vi "base ex info array formation.vi"(11 "Ex info":T1) -> (0 "Tag":string, 1 "Tag 2":string, 3 "Base Ex info array":string[](array[string]))   [LabVIEW 2018]
panel:
  out "配列":string[](array[string])
  out "文字列":string
  out "Level Composition":string[](array[string])
  out "サイズ":i32
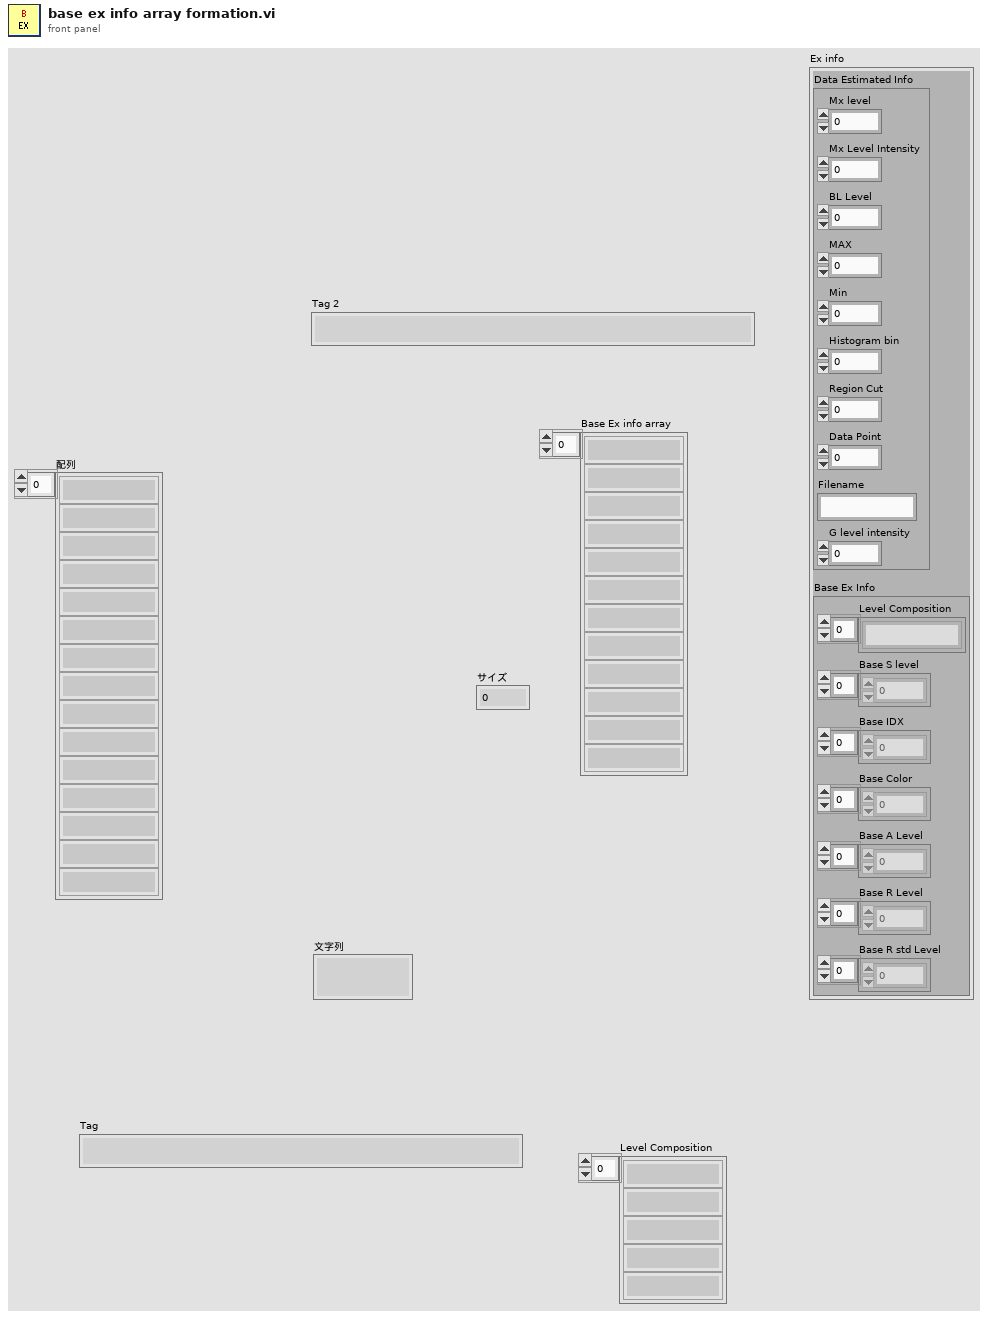
[diagram p1: front panel]
types:
  T1 = cluster{"Data Estimated Info":cluster{"Mx level":dbl, "Mx Level Intensity":dbl, "BL Level":dbl, "MAX":dbl, "Min":dbl, "Histogram bin":dbl, "Region Cut":dbl, "Data Point":i32, "Filename":string, "G level intensity":dbl}, "Base Ex Info":cluster{"Level Composition":string[], "Base S level":dbl[], "Base IDX":i32[], "Base Color":u32[], "Base A Level":dbl[], "Base R Level":dbl[], "Base R std Level":dbl[]}}
  T2 = cluster{"Mx level":dbl, "Mx Level Intensity":dbl, "BL Level":dbl, "MAX":dbl, "Min":dbl, "Histogram bin":dbl, "Region Cut":dbl, "Data Point":i32, "Filename":string, "G level intensity":dbl}
  T3 = cluster{"Level Composition":string[], "Base S level":dbl[], "Base IDX":i32[], "Base Color":u32[], "Base A Level":dbl[], "Base R Level":dbl[], "Base R std Level":dbl[]}
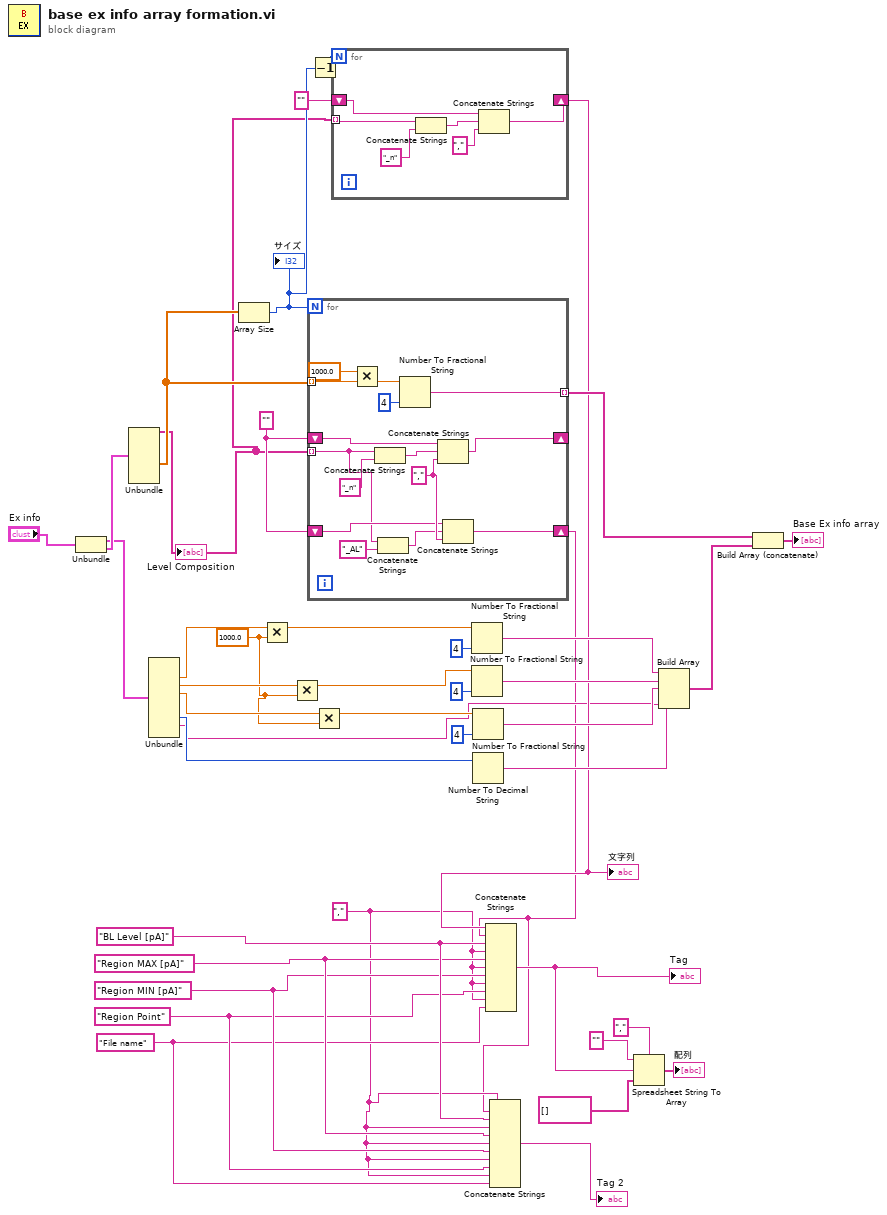
[diagram p0: block diagram]
diagram:
  w6 = "File name" ("書き込みバッファ")
  w13 = 1000.0 ("y")
  w27 = ""
  w7 = "Region Point" ("書き込みバッファ")
  w8 = "Region MIN [pA]" ("書き込みバッファ")
  w9 = "Region MAX [pA]" ("書き込みバッファ")
  w5 = "," ("デリミタ（タブ）")
  w10 = "BL Level [pA]" ("書き込みバッファ")
  n1 = Unbundle("Ex info") -> ("Data Estimated Info"=w1:T2, "Base Ex Info"=w2:T3)
  n2 = Unbundle(w2) -> ("Level Composition"=w19:string[], "Base A Level"=w28:dbl[])  [unwired: 5 out]
  "Level Composition" <- w19
  n3 = Unbundle(w1) -> ("BL Level"=w39:dbl, "MAX"=w35:dbl, "Min"=w33:dbl, "Data Point"=w31:i32, "Filename"=w12:string)  [unwired: 5 out]
  n4 = Array Size(array=w28) -> (size(s)=w21:i32)
  "サイズ" <- w21
  n5 = Multiply(x=w39, y=w13) -> (x*y=w16:dbl)
  n6 = Multiply(x=w35, y=w13) -> (x*y=w15:dbl)
  n7 = for {
    N: w21 -> [_]
    tunnel: w28 -> [w57] mode=indexing
    tunnel: [w55] -> w42 mode=indexing
    tunnel: w19 -> [w45] mode=indexing
    shift-right: [w54] -> _
    shift-left: w27 -> [w48]
    shift-right: [w50] -> w4
    shift-left: w27 -> [w49]
    w51 = "," ("デリミタ（タブ）")
    n8 = Multiply(x=1000.0, y=w57) -> (x*y=w44:dbl)
    n9 = Concatenate Strings(w45, "_n" ("文字列")) -> (w53:string)
    n10 = Concatenate Strings(w45, "_AL" ("文字列")) -> (w47:string)
    n11 = Number To Fractional String(number=w44, precision (6)=i16 4 ("精度（6）")) -> (F-format string=w55:string)  [unwired: 2 in]
    n12 = Concatenate Strings(w48, w53, w51) -> (w54:string)
    n13 = Concatenate Strings(w49, w47, w51) -> (w50:string)
  }
  n14 = Decrement(x=w21) -> (x-1=w20:i32)
  n15 = Multiply(x=w33, y=w13) -> (x*y=w14:dbl)
  n16 = for {
    N: w20 -> [_]
    tunnel: w19 -> [w59] mode=indexing
    shift-right: [w61] -> w17
    shift-left: "" -> [w60]
    n17 = Concatenate Strings(w59, "_n" ("文字列")) -> (w63:string)
    n18 = Concatenate Strings(w60, w63, "," ("デリミタ（タブ）")) -> (w61:string)
  }
  "文字列" <- w17
  n19 = Number To Fractional String(number=w16, precision (6)=i16 4 ("精度（6）")) -> (F-format string=w38:string)  [unwired: 2 in]
  n20 = Number To Fractional String(number=w15, precision (6)=i16 4 ("精度（6）")) -> (F-format string=w34:string)  [unwired: 2 in]
  n21 = Number To Fractional String(number=w14, precision (6)=i16 4 ("精度（6）")) -> (F-format string=w32:string)  [unwired: 2 in]
  n22 = Number To Decimal String(number=w31) -> (decimal integer string=w30:string)  [unwired: 1 in]
  n23 = Concatenate Strings(w17, w4, w10, w5, w9, w5, w8, w5, w7, w5, w6) -> (w26:string)
  "Tag" <- w26
  n24 = Concatenate Strings(w5, w4, w10, w5, w9, w5, w8, w5, w7, w5, w6) -> (→"Tag 2":string)
  n25 = Spreadsheet String To Array(delimiter (Tab)="," ("デリミタ（タブ）"), format string="" ("形式文字列"), spreadsheet string=w26, array type (2D Dbl)=string[] [] ("行ヘッダ文字列[]")) -> (array=→"配列":string[])
  n26 = Build Array(w38, w34, w32, w30, w12) -> (w41:string[])
  n27 = Build Array (concatenate)(w42, w41) -> (→"Base Ex info array":string[])
